vi "Blue Options--constant.vi"() -> (3 "Options":T1={"Force?"=FALSE, "Ignore List"=["Replace String Constants"], "Only List"=[], "Save(T)?"=TRUE})   [LabVIEW 2026]
doc: "Options for linting with blue."
uses:
  <vilib>/SAS/blue/blue_core/API/Options--cluster.ctl
  <vilib>/SAS/blue/blue_core/API/API.lvclass
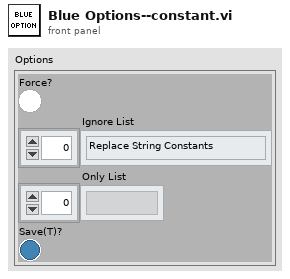
[diagram p1: front panel]
types:
  T1 = typedef "lib_blue_core.lvlib/API.lvclass/Options--cluster.ctl" = cluster{"Force?":bool, "Ignore List":string[], "Only List":string[], "Save(T)?":bool}
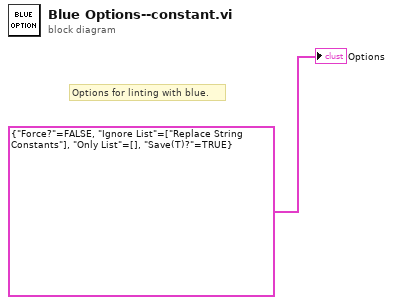
[diagram p0: block diagram]
diagram:
  # "Options for linting with blue."
  "Options" <- T1 {"Force?"=FALSE, "Ignore List"=["Replace String Constants"], "Only List"=[], "Save(T)?"=TRUE} ("Options")
